vi "GO alertes vide.vi"(5 "Numéro":u8) -> ()   [LabVIEW 2022 SP3]
uses:
  Enum/Enum s1.ctl
  Variables globales/Variable glob generale.vi
  Variables globales/Variable glob alertes pressions.vi
  Variables globales/Variable glob mails.vi
  Variables globales/Variable glob Edwards.vi
  Variables globales/Variable glob Leybold.vi
panel:
  out "défautmax pression":bool
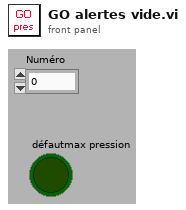
[diagram p1: front panel]
types:
  T1 = typedef "Enum s1.ctl" = enum16{"Alerte vide", "Alerte temperature min-max", "Alerte temperature ecart", "Alerte Keller", "Alerte compteur", "Alerte régulateurs"}
  T2 = cluster{"Alerte":bool, "valeur ":dbl, "Défaut":bool, "Indices controler":i16[], "N°":u16}[]
  T3 = cluster{"Alerte":bool, "valeur ":dbl, "Défaut":bool, "Indices controler":i16[], "N°":u16}
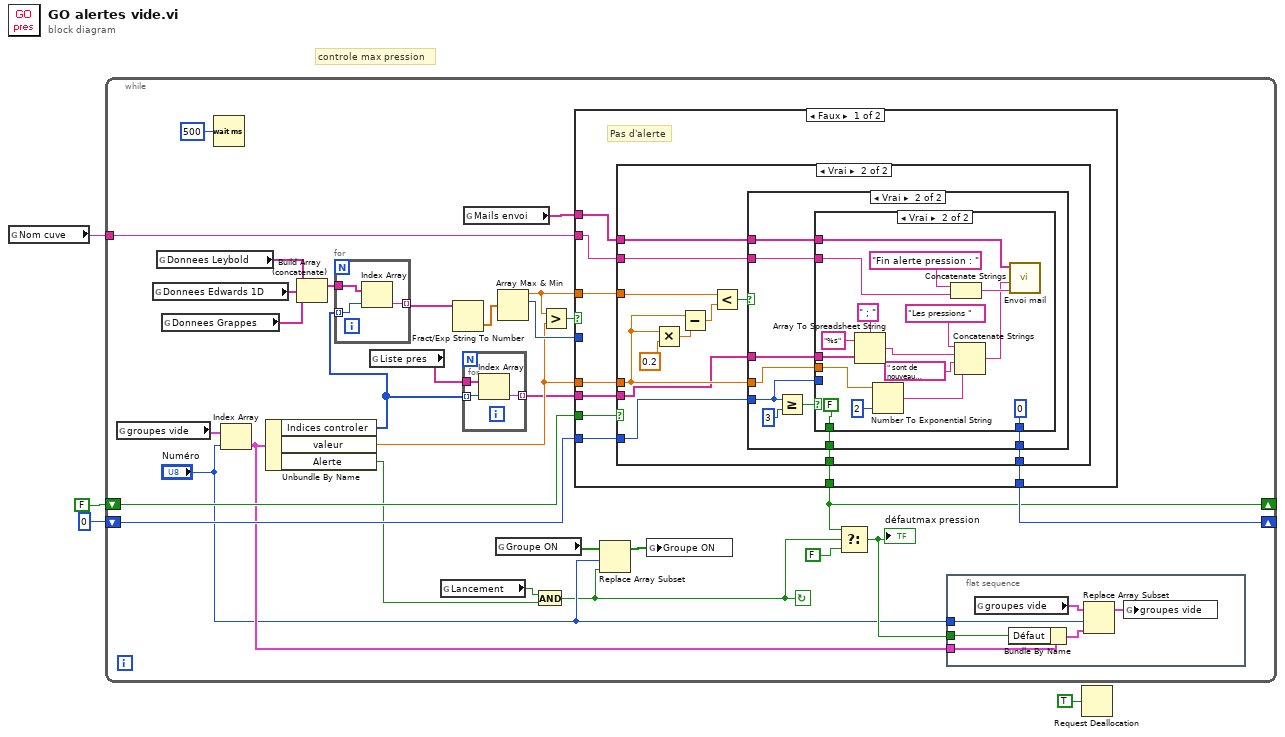
[diagram p0: block diagram]
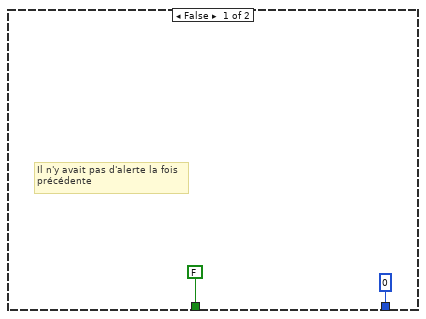
[diagram p2: hidden frame]
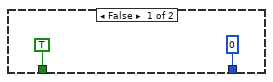
[diagram p3: hidden frame]
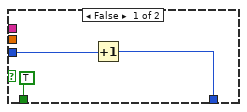
[diagram p4: hidden frame]
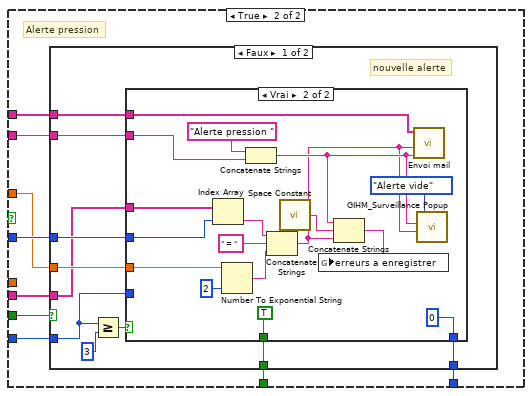
[diagram p5: hidden frame]
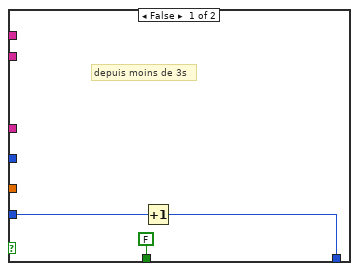
[diagram p6: hidden frame]
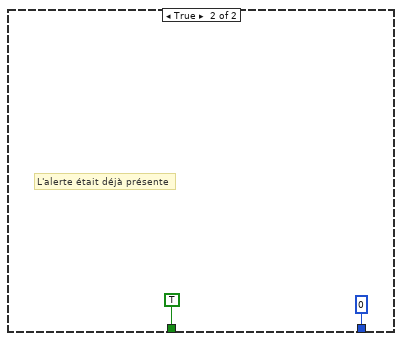
[diagram p7: hidden frame]
diagram:
  # "controle max pression"
  n1 = global read "Variable glob generale.vi" "Nom cuve"() -> (w3:string)
  n2 = while {
    tunnel: w3 -> [w33]
    shift-right: [w21] -> _
    shift-left: FALSE -> [w32]
    shift-right: [w23] -> _
    shift-left: 0 -> [w24]
    stop <- w6 continue-if-true
    n3 = global read "Variable glob alertes pressions.vi" "groupes vide"() -> (w18:T2)
    n4 = global read "Variable glob Edwards.vi" "Donnees Edwards 1D"() -> (w27:string[])
    n5 = global read "Variable glob Leybold.vi" "Donnees Leybold"() -> (w28:string[])
    n6 = global read "Variable glob Edwards.vi" "Donnees Grappes"() -> (w14:string[])
    n7 = Wait (ms)(milliseconds to wait=u32 500 ("attente (ms)")) -> ()  [unwired: 1 out]
    n8 = Index Array(array=w18, index="Numéro") -> (element=w16:T3)
    n9 = Unbundle By Name(w16) -> ("Indices controler"=w10:i16[], "valeur"=w17:dbl, "Alerte"=w13:bool)
    n10 = Build Array (concatenate)(w28, w27, w14) -> (w26:string[])
    n11 = for {
      tunnel: w26 -> [w139]
      tunnel: w10 -> [w140] mode=indexing
      tunnel: [w138] -> w34 mode=indexing
      n12 = Index Array(array=w139, index=w140) -> (element=w138:string)
    }
    n13 = global read "Variable glob alertes pressions.vi" "Liste pres"() -> (w11:string[])
    n14 = global read "Variable glob generale.vi" "Lancement"() -> (w20:bool)
    n15 = Fract/Exp String To Number(string=w34) -> (number=w25:dbl[])  [unwired: 3 in, 1 out]
    n16 = for {
      tunnel: w11 -> [w37]
      tunnel: w10 -> [w36] mode=indexing
      tunnel: [w35] -> w9 mode=indexing
      n17 = Index Array(array=w37, index=w36) -> (element=w35:string)
    }
    n18 = global read "Variable glob mails.vi" "Mails envoi"() -> (w12:string[])
    n19 = global read "Variable glob alertes pressions.vi" "Groupe ON"() -> (w8:bool[])
    n20 = Array Max & Min(array=w25) -> (max value=w30:dbl, max index (indices)=w31:i32)  [unwired: 2 out]
    n21 = And(x=w20, y=w13) -> (x .and. y?=w6:bool)
    n22 = Greater?(x=w30, y=w17) -> (0:w29:bool)
    n23 = case shown="Faux" w29 {
      tunnel: w33 -> [w52 w105]
      tunnel: w32 -> [w50 w104]
      tunnel: w31 -> [_ w103]
      tunnel: w30 -> [w47 w102]
      tunnel: w17 -> [w51 _]
      tunnel: w12 -> [w49 w101]
      tunnel: [w48 w100] -> w21
      tunnel: w24 -> [w46 w99]
      tunnel: [w45 w98] -> w23
      tunnel: w9 -> [w44 w97]
      frame False {
        # "Pas d'alerte"
        n24 = case shown="Vrai" w50 {
          tunnel: w51 -> [_ w62]
          tunnel: w52 -> [_ w65]
          tunnel: w49 -> [_ w66]
          tunnel: [FALSE w57] -> w48
          tunnel: w47 -> [_ w64]
          tunnel: w46 -> [_ w58]
          tunnel: [0 w59] -> w45
          tunnel: w44 -> [_ w55]
          frame False {
            # "Il n'y avait pas d'alerte la fois\nprécédente"
          }
          frame True {
            n25 = Multiply(x=w62, y=0.2) -> (x*y=w60:dbl)
            n26 = Subtract(x=w62, y=w60) -> (x-y=w63:dbl)
            n27 = Less?(x=w64, y=w63) -> (x < y?=w56:bool)
            n28 = case shown="Vrai" w56 {
              tunnel: w62 -> [_ w77]
              tunnel: w66 -> [_ w76]
              tunnel: w65 -> [_ w75]
              tunnel: [0 w74] -> w59
              tunnel: w58 -> [_ w70]
              tunnel: [TRUE w73] -> w57
              tunnel: w55 -> [_ w69]
              frame False {
              }
              frame True {
                n29 = Greater Or Equal?(x=w70, y=3) -> (x >= y?=w71:bool)
                n30 = case shown="Vrai" w71 {
                  tunnel: w77 -> [_ w96]
                  tunnel: w76 -> [_ w92]
                  tunnel: w75 -> [_ w91]
                  tunnel: [w78 0] -> w74
                  tunnel: [TRUE FALSE] -> w73
                  tunnel: w70 -> [w79 _]
                  tunnel: w69 -> [_ w86]
                  frame False {
                    n31 = Increment(x=w79) -> (x+1=w78:i32)
                  }
                  frame True {
                    n32 = Array To Spreadsheet String(delimiter (Tab)=" ; " ("séparateur (Tabulation)"), array=w86, 3:"%s" ("chaîne de format")) -> (spreadsheet string=w83:string)
                    n33 = Number To Exponential String(number=w96, precision (6)=i16 2 ("précision (6)")) -> (E-format string=w81:string)  [unwired: 2 in]
                    n34 = Concatenate Strings("Fin alerte pression : " ("subject ([No Subject])"), w91) -> (w90:string)
                    n35 = Concatenate Strings("Les pressions ", w83, " sont de nouveau inférieures à ", w81) -> (w89:string)
                    n36 = call "Envoi mail.vi"("Objet"=w90, "Message"=w89, "Mail liste"=w92) -> ()  [unwired: 3 in]
                  }
                }
              }
            }
          }
        }
      }
      frame True {
        # "Alerte pression"
        n37 = case shown="Faux" w104 {
          tunnel: w105 -> [w112 _]
          tunnel: w103 -> [w115 _]
          tunnel: w102 -> [w114 _]
          tunnel: w101 -> [w113 _]
          tunnel: [w111 TRUE] -> w100
          tunnel: w99 -> [w108 _]
          tunnel: [w107 0] -> w98
          tunnel: w97 -> [w106 _]
          frame False {
            # "nouvelle alerte"
            n38 = Greater Or Equal?(x=w108, y=3) -> (x >= y?=w109:bool)
            n39 = case shown="Vrai" w109 {
              tunnel: w115 -> [_ w132]
              tunnel: w114 -> [_ w131]
              tunnel: w113 -> [_ w128]
              tunnel: w112 -> [_ w127]
              tunnel: [FALSE TRUE] -> w111
              tunnel: w108 -> [w117 _]
              tunnel: [w116 0] -> w107
              tunnel: w106 -> [_ w122]
              frame False {
                # "depuis moins de 3s"
                n40 = Increment(x=w117) -> (x+1=w116:i32)
              }
              frame True {
                n41 = Index Array(array=w122, index=w132) -> (element=w133:string)
                n42 = Number To Exponential String(number=w131, precision (6)=i16 2 ("précision (6)")) -> (E-format string=w134:string)  [unwired: 2 in]
                n43 = Concatenate Strings("Alerte pression " ("subject ([No Subject])"), w127) -> (w121:string)
                n44 = Concatenate Strings(w133, " = " ("chaîne"), w134) -> (w120:string)
                n45 = call <vilib>:"Space Constant.vi"() -> ("String"=w123:string)
                n46 = Concatenate Strings(w121, w123, w120) -> (w124:string)
                n47 = global write "Variable glob generale.vi" "erreurs a enregistrer"(w124) -> ()
                n48 = call "Envoi mail.vi"("Objet"=w121, "Message"=w120, "Mail liste"=w128) -> ()  [unwired: 3 in]
                n49 = call "GIHM_Surveillance Popup.vi"("Message"=w120, "Problème observé"=w121, "Type problème"=Enum_s1."Alerte vide") -> ()  [unwired: 2 in, 1 out]
              }
            }
          }
          frame True {
            # "L'alerte était déjà présente"
          }
        }
      }
    }
    n50 = Replace Array Subset(array=w8, new element=w6, index="Numéro") -> (w5:bool[])
    n51 = global write "Variable glob alertes pressions.vi" "Groupe ON"(w5) -> ()
    n52 = Select(t=w21, s=w6, f=FALSE ("cas faux")) -> (s? t:f=w15:bool)
    "défautmax pression" <- w15
    n53 = flat-sequence {
      tunnel: "Numéro" -> [w42]
      tunnel: w16 -> [w41]
      tunnel: w15 -> [w38]
      frame #0 {
        n54 = global read "Variable glob alertes pressions.vi" "groupes vide"() -> (w43:T2)
        n55 = Bundle By Name(cluster=w41, "Défaut"=w38) -> (w40:T3)
        n56 = Replace Array Subset(array=w43, new element=w40, index=w42) -> (w39:T2)
        n57 = global write "Variable glob alertes pressions.vi" "groupes vide"(w39) -> ()
      }
    }
  }
  n58 = Request Deallocation(TRUE ("flag")) -> ()
